vi "SC Pick Deploy.vi"(4 "projects":T1(array[cluster]), 5 "copy":string, 6 "local":i32=-1, 7 "struck":bool[](array[boolean]), 8 "symbols":i32[](array[numeric]), 9 "items":string[](array[string]), 10 "window title":string="Deploy History", 11 "current":i32=-1) -> (0 "project":i32=-1, 1 "index":i32=-1, 2 "chosen?":bool, 3 "action":string)   [LabVIEW 2023]
doc: "Shows a window listing the items, each with its symbol, the current one in bold, the local one in italics and struck ones struck through, with Check Out, Redeploy and Cancel buttons. Double-clicking an item or selecting it and clicking Redeploy returns its index; action is redeploy or check out (with chosen? and index), delete project (the Delete Project button), open copy (Open Project, shown when copy names the shown project's local .lvproj), fetch project (Fetch Project, shown instead of Delete Project when there's no local copy), or empty. chosen? is false when the user cancels or closes the window."
panel:
  in  "Fetch Project":bool
  in  "Open Project":bool
  in  "Delete Project":bool
  in  "Project":u16(ring)
  in  "Check Out":bool
  in  "Cancel":bool
  in  "Redeploy":bool
  in  "Deploys":i32(listbox)=-1
  out "check out?":bool
  out "delete project?":bool
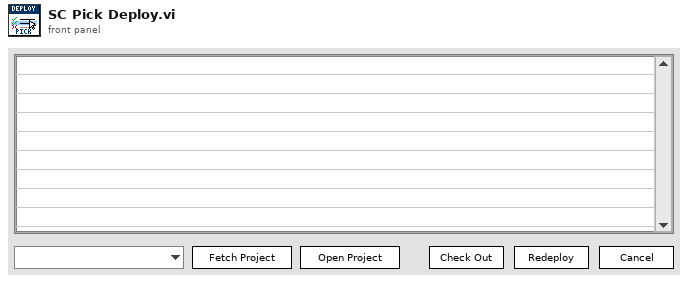
[diagram p1: front panel]
types:
  T1 = cluster{"name":string, "running":bool, "local copy":bool}[]
  T2 = typedef "LVRectTypeDef.ctl" = cluster{"Left":i16, "Top":i16, "Right":i16, "Bottom":i16}
  T3 = typedef "LVPositionTypeDef.ctl" = cluster{"Left":i32, "Top":i32}
  T4 = cluster{"name":string, "running":bool, "local copy":bool}
  T5 = typedef "LVPoint32TypeDef.ctl" = cluster{"Horizontal":i32, "Vertical":i32}
  T6 = typedef "LVRowAndColumnTypeDef.ctl" = cluster{"Row":i32, "Column":i32}
  T7 = typedef "LVPointTypeDef.ctl" = cluster{"Horizontal":i16, "Vertical":i16}
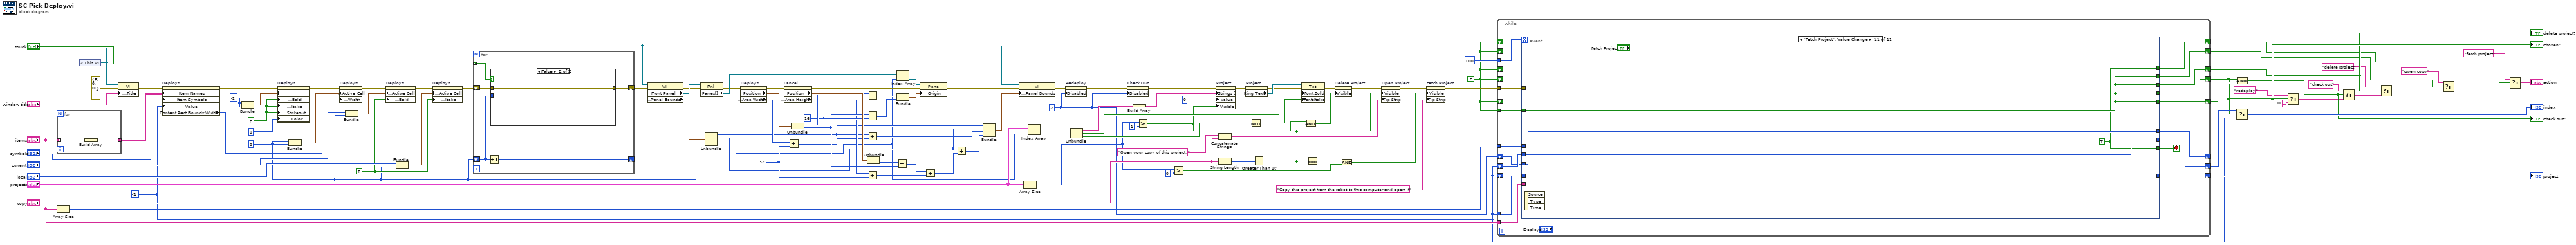
[diagram p0: block diagram]
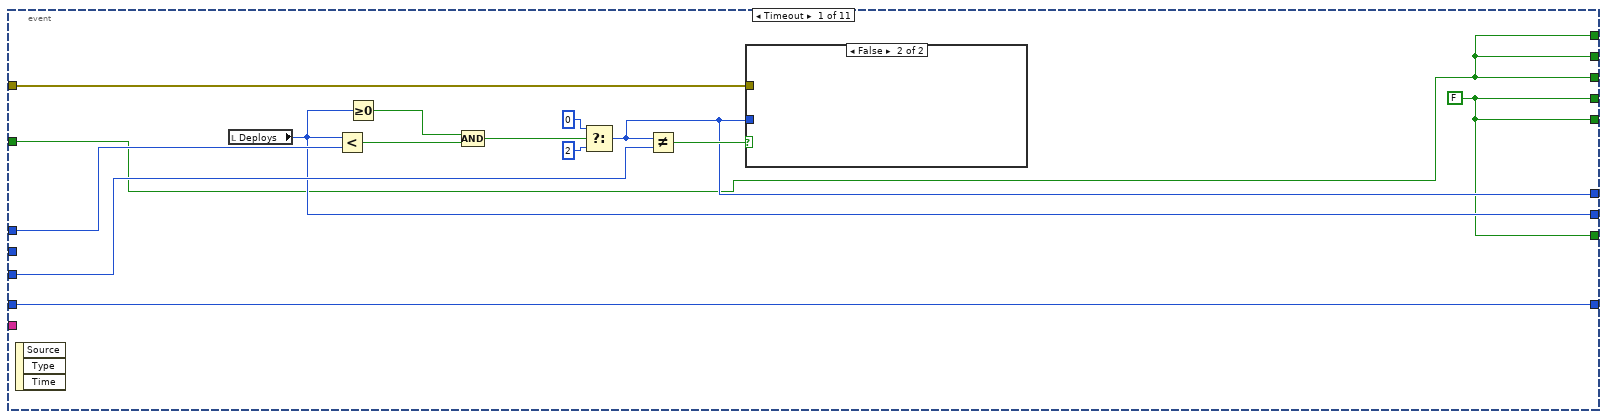
[diagram p2: hidden frame]
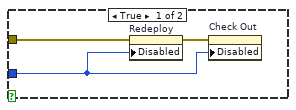
[diagram p3: hidden frame]
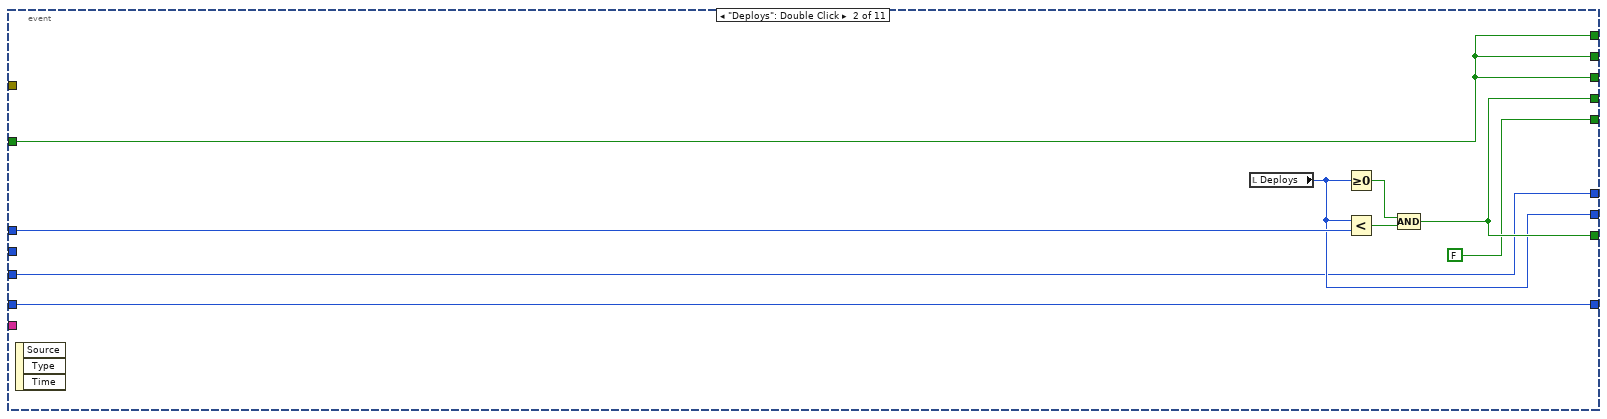
[diagram p4: hidden frame]
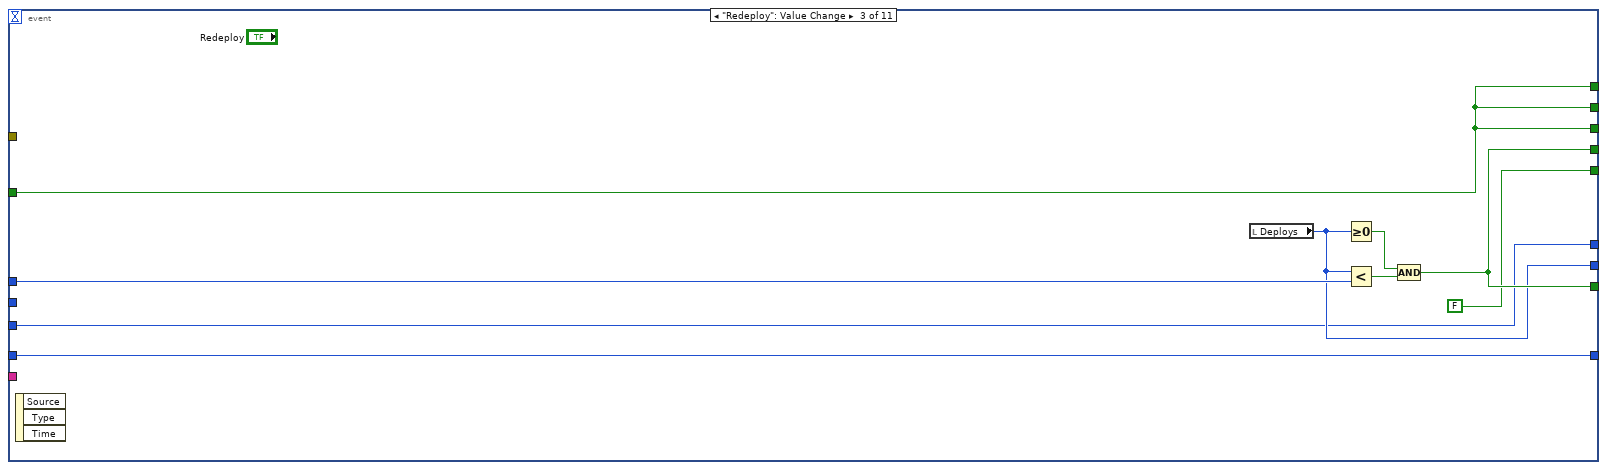
[diagram p5: hidden frame]
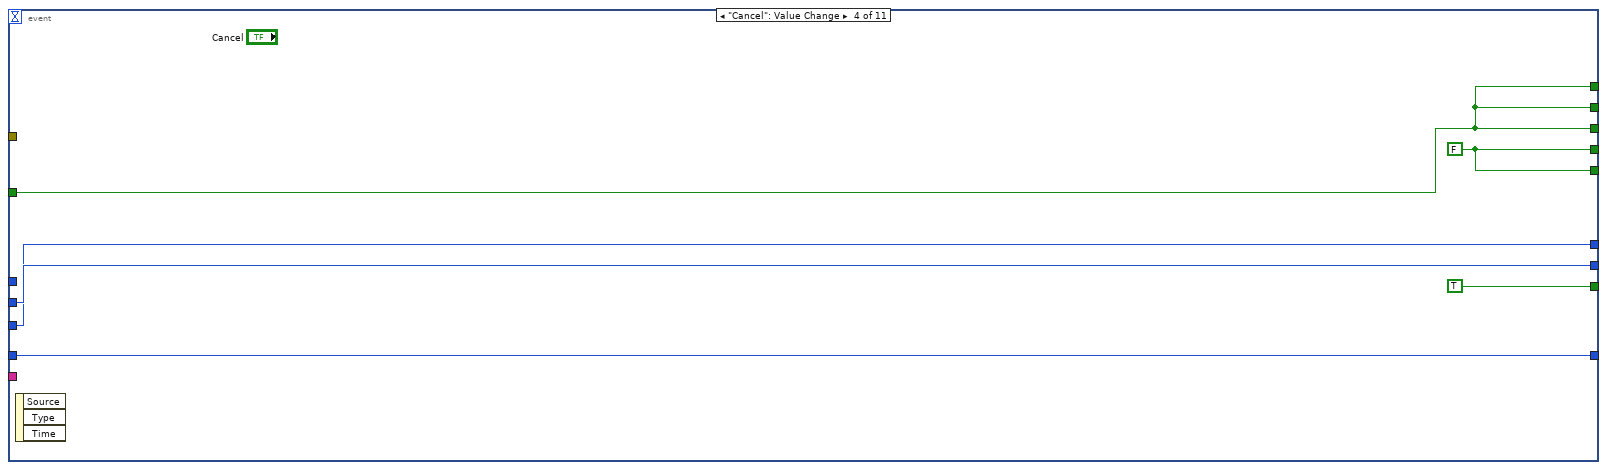
[diagram p6: hidden frame]
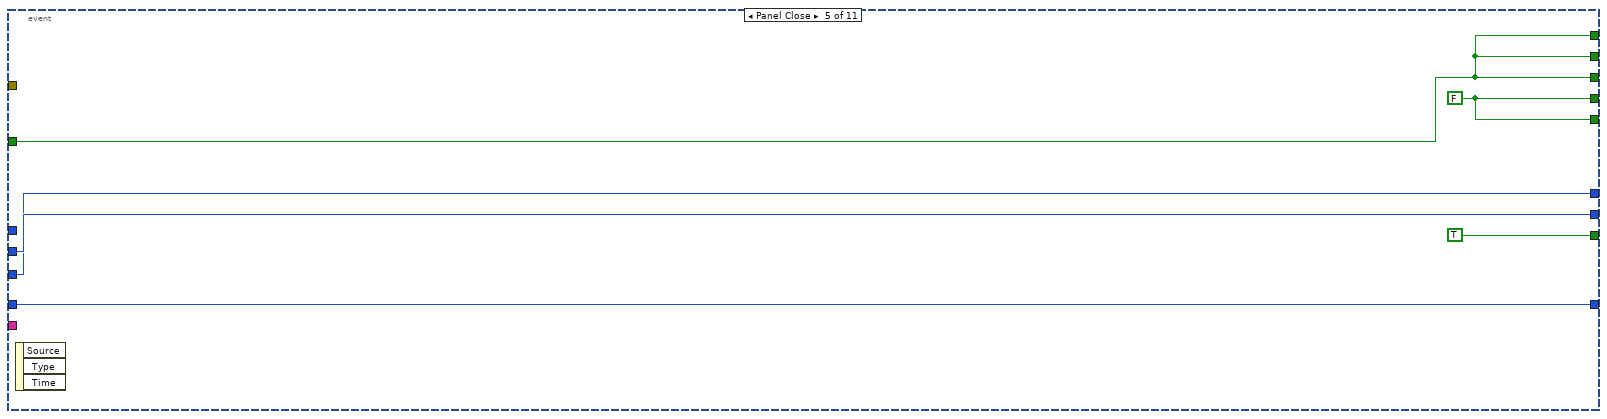
[diagram p7: hidden frame]
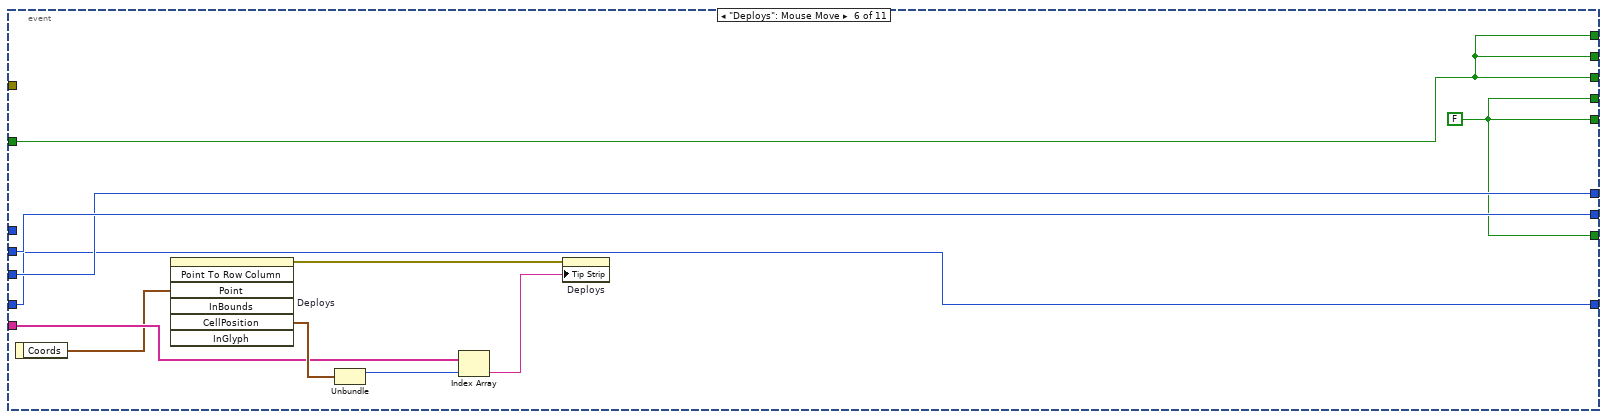
[diagram p8: hidden frame]
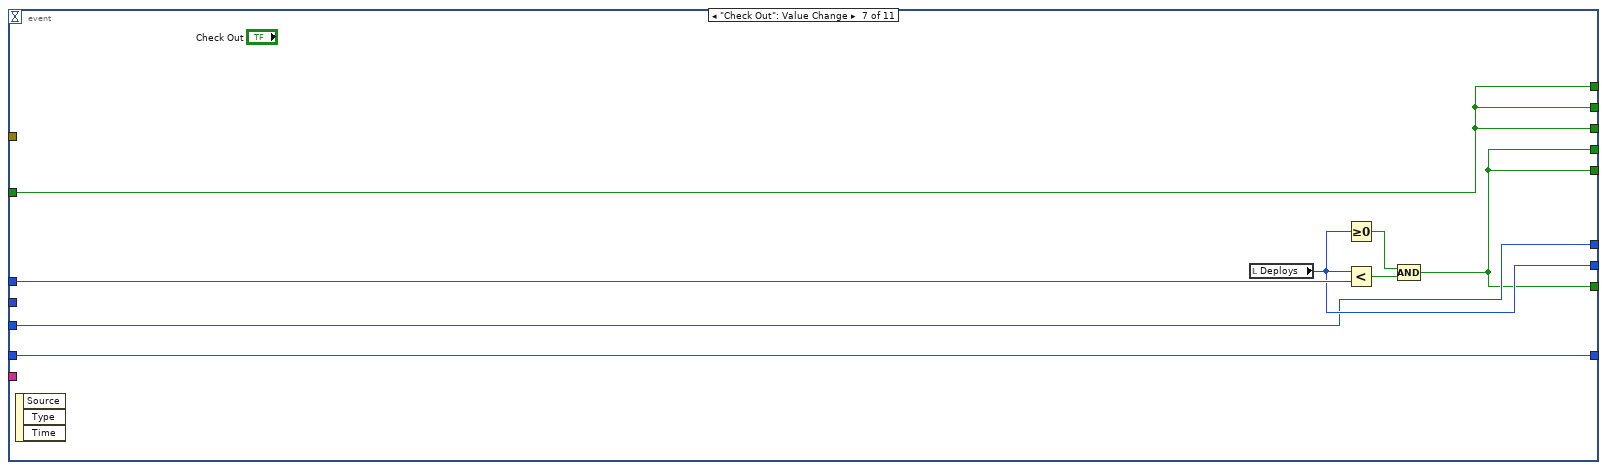
[diagram p9: hidden frame]
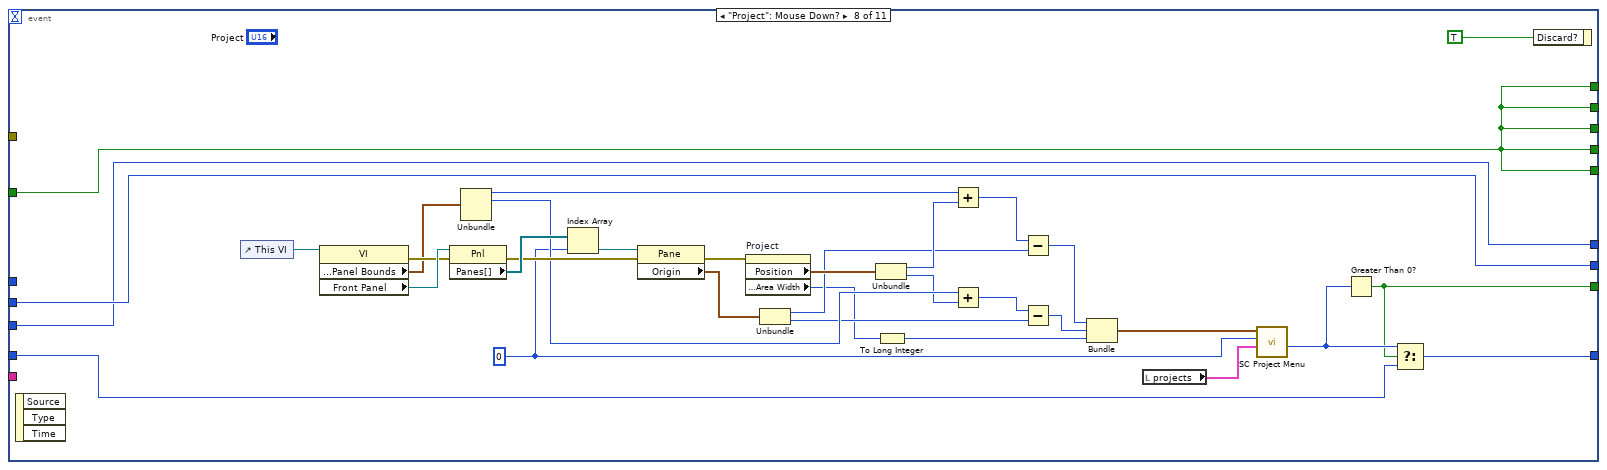
[diagram p10: hidden frame]
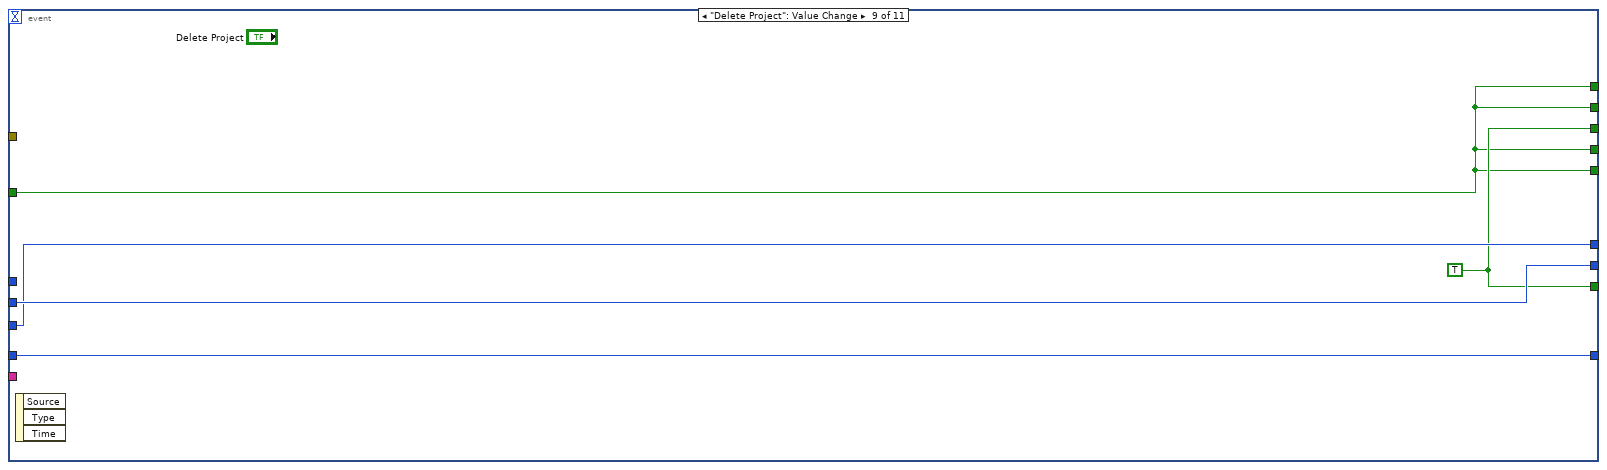
[diagram p11: hidden frame]
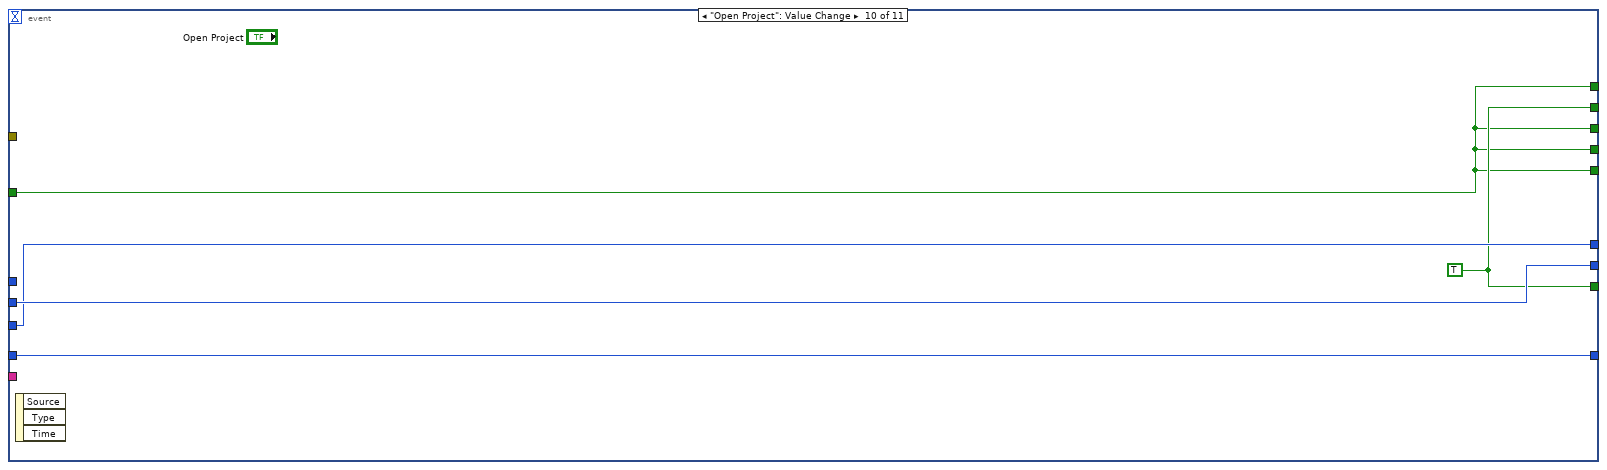
[diagram p12: hidden frame]
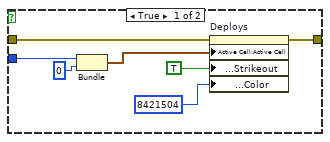
[diagram p13: hidden frame]
diagram:
  w22 = FALSE
  w74 = 32
  w81 = 16
  w94 = TRUE
  w55 = 0
  w105 = FALSE
  w108 = -2
  w21 = u8 2
  w19 = -1
  n1 = for {
    tunnel: "items" -> [w115] mode=indexing
    tunnel: [w114] -> w110 mode=indexing
    n2 = Build Array(w115) -> (w114:string[])
  }
  n3 = Array Size(array="items") -> (size(s)=w27:i32)
  n4 = control-ref of="This VI"() -> (w62:refnum<vi>)
  n5 = property class="VI"(reference=w62, error in=errorcluster {"status"=FALSE, "code"=0, "source"=""}, "Front Panel Window:Title"="window title") -> (error out=w111:errorcluster)  [unwired: 1 out]
  n6 = property on="Deploys" class="MCListbox (strict)"(error in=w111, "Item Names"=w110, "Item Symbols"="symbols", "Value"=w19) -> (error out=w107:errorcluster, "Content Rect Bounds:Width"=w100:i32)  [unwired: 1 in, 1 out]
  n7 = Bundle(w108, w108) -> (w106:cluster{i32, i32})  [unwired: 1 in]
  n8 = property on="Deploys" class="MCListbox (strict)"(error in=w107, "Active Cell:Active Cell"=w106, "Active Cell:Cell Font:Bold"=w105, "Active Cell:Cell Font:Italic"=w105, "Active Cell:Cell Font:Strikeout"=w105, "Active Cell:Cell Font:Color"=u32 0) -> (error out=w102:errorcluster)  [unwired: 1 in, 1 out]
  n9 = Bundle(w55, w55) -> (w101:cluster{i32, i32})  [unwired: 1 in]
  n10 = property on="Deploys" class="MCListbox (strict)"(error in=w102, "Active Cell:Active Cell"=w101, "Active Cell:Cell Size:Width"=w100) -> (error out=w99:errorcluster)  [unwired: 1 in, 1 out]
  n11 = Bundle("current"="current", w55) -> (w98:cluster{"current":i32, i32})  [unwired: 1 in]
  n12 = property on="Deploys" class="MCListbox (strict)"(error in=w99, "Active Cell:Active Cell"=w98, "Active Cell:Cell Font:Bold"=w94) -> (error out=w96:errorcluster)  [unwired: 1 in, 1 out]
  n13 = Bundle("local"="local", w55) -> (w95:cluster{"local":i32, i32})  [unwired: 1 in]
  n14 = property on="Deploys" class="MCListbox (strict)"(error in=w96, "Active Cell:Active Cell"=w95, "Active Cell:Cell Font:Italic"=w94) -> (error out=w92:errorcluster)  [unwired: 1 in, 1 out]
  n15 = for {
    tunnel: "struck" -> [w116] mode=indexing
    shift-right: [w120] -> _
    shift-left: w55 -> [w119]
    shift-right: [w117] -> w91
    shift-left: w92 -> [w118]
    n16 = Increment(x=w119) -> (x+1=w120:i32)
    n17 = case shown="False" w116 {
      tunnel: w119 -> [w127 _]
      tunnel: w118 -> [w125 w128]
      tunnel: [w121 w128] -> w117
      frame True {
        n18 = Bundle(w127, 0) -> (w124:cluster{i32, i32})  [unwired: 1 in]
        n19 = property on="Deploys" class="MCListbox (strict)"(error in=w125, "Active Cell:Active Cell"=w124, "Active Cell:Cell Font:Strikeout"=TRUE, "Active Cell:Cell Font:Color"=u32 8421504) -> (error out=w121:errorcluster)  [unwired: 1 in, 1 out]
      }
      frame False {
      }
    }
  }
  n20 = property class="VI"(reference=w62, error in=w91) -> (error out=w89:errorcluster, "Front Panel"=w90:refnum<vi>, "Front Panel Window:Panel Bounds"=w83:T2)  [unwired: 1 out]
  n21 = property class="Pnl"(reference=w90, error in=w89) -> (error out=w87:errorcluster, "Panes[]"=w88:refnum<vi>[])  [unwired: 1 out]
  n22 = Unbundle(w83) -> ("Left"=w69:i16, "Top"=w68:i16)  [unwired: 2 out]
  n23 = property on="Deploys" class="MCListbox (strict)"(error in=w87) -> (error out=w86:errorcluster, "Position"=w85:T3, "Bounds:Area Width"=w78:u32)  [unwired: 1 in, 1 out]
  n24 = property on="Cancel" class="Bool"(error in=w86) -> (error out=w64:errorcluster, "Position"=w84:T3, "Bounds:Area Height"=w75:u32)  [unwired: 1 in, 1 out]
  n25 = Add(x=w78, y=w74) -> (x+y=w71:u32)
  n26 = Unbundle(w85) -> ("Left"=w82:i32, "Top"=w76:i32)
  n27 = Subtract(x=w82, y=w81) -> (x-y=w80:i32)
  n28 = Subtract(x=w76, y=w81) -> (x-y=w79:i32)
  n29 = Add(x=w69, y=w71) -> (x+y=w67:u32)
  n30 = Add(x=w75, y=w74) -> (x+y=w72:u32)
  n31 = Unbundle(w84) -> ("Top"=w77:i32)  [unwired: 1 out]
  n32 = Subtract(x=w77, y=w76) -> (x-y=w73:i32)
  n33 = Index Array(array=w88, index=w55) -> (element=w65:refnum<vi>)
  n34 = Bundle(w80, w79) -> (w63:cluster{i32, i32})  [unwired: 1 in]
  n35 = property class="Pane"(reference=w65, error in=w64, "Origin"=w63) -> (error out=w61:errorcluster)  [unwired: 1 out]
  n36 = Add(x=w73, y=w72) -> (x+y=w70:u32)
  n37 = Add(x=w68, y=w70) -> (x+y=w66:u32)
  n38 = Bundle("Left"=w69, "Top"=w68, w67, w66) -> (w60:cluster{"Left":i16, "Top":i16, u32, u32})  [unwired: 1 in]
  n39 = property class="VI"(reference=w62, error in=w61, "Front Panel Window:Panel Bounds"=w60) -> (error out=w59:errorcluster)  [unwired: 1 out]
  n40 = Array Size(array="projects") -> (size(s)=w34:i32)
  n41 = Index Array(array="projects", index=w55) -> (element=w54:T4)
  n42 = property on="Redeploy" class="Bool"(error in=w59, "Disabled"=w21) -> (error out=w58:errorcluster)  [unwired: 1 in, 1 out]
  n43 = Unbundle(w54) -> ("name"=w53:string, "running"=w49:bool, "local copy"=w52:bool)
  n44 = property on="Check Out" class="Bool"(error in=w58, "Disabled"=w21) -> (error out=w47:errorcluster)  [unwired: 1 in, 1 out]
  n45 = Build Array(w53) -> (w46:string[])
  n46 = Greater?(x=w34, y=1) -> (0:w37:bool)
  n47 = Greater?(x=w34, y=0) -> (0:w31:bool)
  n48 = property on="Project" class="Ring (strict)"(error in=w47, "Strings []"=w46, "Value"=u16 0, "Visible"=w37) -> (error out=w44:errorcluster)  [unwired: 1 in, 1 out]
  n49 = Concatenate Strings("Open your copy of this project: ", "copy") -> (w38:string)
  n50 = String Length(string="copy") -> (length=w42:i32)
  n51 = property on="Project" class="Ring (strict)"(error in=w44) -> (error out=w50:errorcluster, "Ring Text"=w51:refnum<vi>)  [unwired: 1 in, 1 out]
  n52 = Not(x=w52) -> (.not. x?=w48:bool)
  n53 = Greater Than 0?(x=w42) -> (x > 0?=w35:bool)
  n54 = property class="Txt"(reference=w51, error in=w50, "Font:Bold"=w49, "Font:Italic"=w48) -> (error out=w43:errorcluster)  [unwired: 1 out]
  n55 = And(x=w37, y=w35) -> (x .and. y?=w36:bool)
  n56 = Not(x=w35) -> (.not. x?=w32:bool)
  n57 = property on="Delete Project" class="Bool"(error in=w43, "Visible"=w36) -> (error out=w39:errorcluster)  [unwired: 1 in, 1 out]
  n58 = And(x=w32, y=w31) -> (x .and. y?=w29:bool)
  n59 = property on="Open Project" class="Bool"(error in=w39, "Visible"=w35, "Tip Strip"=w38) -> (error out=w30:errorcluster)  [unwired: 1 in, 1 out]
  n60 = property on="Fetch Project" class="Bool"(error in=w30, "Visible"=w29, "Tip Strip"="Copy this project from the robot to this computer and open it") -> (error out=w26:errorcluster)  [unwired: 1 in, 1 out]
  n61 = while {
    tunnel: w27 -> [w145]
    tunnel: w26 -> [w143]
    tunnel: 100 -> [w129]
    tunnel: "items" -> [w141]
    tunnel: w19 -> [w137]
    tunnel: w22 -> [w136]
    shift-right: [w139] -> w20
    shift-left: w19 -> [w144]
    shift-right: [w140] -> w16
    shift-left: w22 -> [_]
    shift-right: [w135] -> w17
    shift-left: w22 -> [_]
    shift-right: [w134] -> w23
    shift-left: w19 -> [_]
    shift-right: [w133] -> w10
    shift-left: w22 -> [_]
    shift-right: [w131] -> w4
    shift-left: w22 -> [_]
    shift-right: [w132] -> w7
    shift-left: w22 -> [_]
    shift-right: [w138] -> _
    shift-left: w21 -> [w142]
    stop <- w130 stop-if-true
    n62 = event shown="[10] \"Fetch Project\": Value Change" {
      selector: _ -> [_ _ _ _ _ _ _ _ _ _ _]
      dyn-events: _ -> [_ _ _ _ _ _ _ _ _ _ _]
      timeout: w129 -> [_ _ _ _ _ _ _ _ _ _ _]
      tunnel: w145 -> [w159 w171 w180 _ _ _ w211 _ _ _ _]
      tunnel: w144 -> [_ _ _ w185 w191 w198 _ w216 w249 w254 w259]
      tunnel: w143 -> [w152 _ _ _ _ _ _ _ _ _ _]
      tunnel: w142 -> [w153 w166 w175 w184 w190 w197 w207 w215 w248 w253 w258]
      tunnel: w141 -> [_ _ _ _ _ w202 _ _ _ _ _]
      tunnel: [w148 w168 w177 TRUE TRUE w196 w206 w217 w246 w251 w255] -> w130
      tunnel: [w148 w168 w177 w183 w189 w196 w206 w213 w245 w250 w256] -> w140
      tunnel: [w150 w167 w176 w185 w191 w198 w208 w216 w249 w254 w259] -> w139
      tunnel: [w149 w166 w175 w184 w190 w197 w207 w215 w248 w253 w258] -> w138
      tunnel: w137 -> [w147 w164 w173 w182 w188 w195 w205 w218 w247 w252 w257]
      tunnel: w136 -> [w146 w163 w172 w181 w187 w194 w204 w213 w245 w250 w256]
      tunnel: [w148 FALSE FALSE w183 w189 w196 w206 w213 w245 w250 w256] -> w135
      tunnel: [w147 w164 w173 w182 w188 w195 w205 w214 w247 w252 w257] -> w134
      tunnel: [w146 w163 w172 w181 w187 w194 w204 w213 w246 w250 w256] -> w133
      tunnel: [w146 w163 w172 w181 w187 w194 w204 w213 w245 w251 w256] -> w132
      tunnel: [w146 w163 w172 w181 w187 w194 w204 w213 w245 w250 w255] -> w131
      event Timeout {
        w148 = FALSE
        n63 = event-data() -> ()  [unwired: 1 in, 3 out]
        n64 = local read "Deploys"() -> (w150:i32)
        n65 = Less?(x=w150, y=w159) -> (x < y?=w157:bool)
        n66 = Greater Or Equal To 0?(x=w150) -> (x >= 0?=w158:bool)
        n67 = Compound Arithmetic op=AND(w158, w157) -> (w156:bool)
        n68 = Select(t=u8 0, s=w156, f=u8 2) -> (s? t:f=w149:u8)
        n69 = Not Equal?(x=w149, y=w153) -> (x != y?=w151:bool)
        n70 = case shown="False" w151 {
          tunnel: w149 -> [w160 _]
          tunnel: w152 -> [w162 _]
          frame True {
            n71 = property on="Redeploy" class="Bool"(error in=w162, "Disabled"=w160) -> (error out=w161:errorcluster)  [unwired: 1 in, 1 out]
            n72 = property on="Check Out" class="Bool"(error in=w161, "Disabled"=w160) -> ()  [unwired: 1 in, 2 out]
          }
          frame False {
          }
        }
      }
      event "Deploys": Double Click {
        n73 = event-data() -> ()  [unwired: 1 in, 3 out]
        n74 = local read "Deploys"() -> (w167:i32)
        n75 = Greater Or Equal To 0?(x=w167) -> (x >= 0?=w170:bool)
        n76 = Less?(x=w167, y=w171) -> (x < y?=w169:bool)
        n77 = Compound Arithmetic op=AND(w170, w169) -> (w168:bool)
      }
      event "Redeploy": Value Change {
        n78 = event-data() -> ()  [unwired: 1 in, 3 out]
        n79 = local read "Deploys"() -> (w176:i32)
        n80 = Greater Or Equal To 0?(x=w176) -> (x >= 0?=w179:bool)
        n81 = Less?(x=w176, y=w180) -> (x < y?=w178:bool)
        n82 = Compound Arithmetic op=AND(w179, w178) -> (w177:bool)
      }
      event "Cancel": Value Change {
        w183 = FALSE
        n83 = event-data() -> ()  [unwired: 1 in, 3 out]
      }
      event Panel Close {
        w189 = FALSE
        n84 = event-data() -> ()  [unwired: 1 in, 3 out]
      }
      event "Deploys": Mouse Move {
        w196 = FALSE
        n85 = event-data() -> ("Coords"=w193:T5)  [unwired: 1 in]
        n86 = invoke on="Deploys" class="MCListbox (strict)" method="Point To Row Column"("Point"=w193) -> (error out=w200:errorcluster, "CellPosition"=w203:T6)  [unwired: 6 in, 5 out]
        n87 = Unbundle(w203) -> ("Row"=w201:i32)  [unwired: 1 out]
        n88 = Index Array(array=w202, index=w201) -> (element=w199:string)
        n89 = property on="Deploys" class="MCListbox (strict)"(error in=w200, "Tip Strip"=w199) -> ()  [unwired: 1 in, 2 out]
      }
      event "Check Out": Value Change {
        n90 = event-data() -> ()  [unwired: 1 in, 3 out]
        n91 = local read "Deploys"() -> (w208:i32)
        n92 = Greater Or Equal To 0?(x=w208) -> (x >= 0?=w210:bool)
        n93 = Less?(x=w208, y=w211) -> (x < y?=w209:bool)
        n94 = Compound Arithmetic op=AND(w210, w209) -> (w206:bool)
      }
      event "Project": Mouse Down? {
        w221 = 0
        n95 = event-data() -> ()  [unwired: 1 in, 3 out]
        n96 = control-ref of="This VI"() -> (w244:refnum<vi>)
        n97 = property class="VI"(reference=w244) -> (error out=w242:errorcluster, "Front Panel Window:Panel Bounds"=w237:T2, "Front Panel"=w243:refnum<vi>)  [unwired: 1 in, 1 out]
        n98 = property class="Pnl"(reference=w243, error in=w242) -> (error out=w239:errorcluster, "Panes[]"=w241:refnum<vi>[])  [unwired: 1 out]
        n99 = Unbundle(w237) -> ("Left"=w234:i16, "Top"=w230:i16)  [unwired: 2 out]
        n100 = Index Array(array=w241, index=w221) -> (element=w240:refnum<vi>)
        n101 = property class="Pane"(reference=w240, error in=w239) -> (error out=w238:errorcluster, "Origin"=w236:T7)  [unwired: 1 out]
        n102 = property on="Project" class="Ring (strict)"(error in=w238) -> ("Position"=w235:T3, "Bounds:Area Width"=w226:u32)  [unwired: 1 in, 2 out]
        n103 = Unbundle(w236) -> ("Horizontal"=w231:i16, "Vertical"=w227:i16)
        n104 = Unbundle(w235) -> ("Left"=w233:i32, "Top"=w229:i32)
        n105 = To Long Integer(number=w226) -> (32bit integer=w223:i32)
        n106 = Add(x=w234, y=w233) -> (x+y=w232:i32)
        n107 = Add(x=w230, y=w229) -> (x+y=w228:i32)
        n108 = Subtract(x=w232, y=w231) -> (x-y=w225:i32)
        n109 = Subtract(x=w228, y=w227) -> (x-y=w224:i32)
        n110 = Bundle(w225, w224, w223) -> (w220:cluster{i32, i32, i32})  [unwired: 1 in]
        n111 = local read "projects"() -> (w222:T1)
        n112 = call "SC Project Menu.vi"("projects"=w222, "selected"=w221, "position"=w220) -> ("index"=w219:i32)  [unwired: 8 in]
        n113 = Greater Than 0?(x=w219) -> (x > 0?=w217:bool)
        n114 = Select(t=w219, s=w217, f=w218) -> (s? t:f=w214:i32)
        n115 = event-data("Discard?"=TRUE) -> ()  [unwired: 1 in, 1 out]
      }
      event "Delete Project": Value Change {
        w246 = TRUE
        n116 = event-data() -> ()  [unwired: 1 in, 3 out]
      }
      event "Open Project": Value Change {
        w251 = TRUE
        n117 = event-data() -> ()  [unwired: 1 in, 3 out]
      }
      event "Fetch Project": Value Change {
        w255 = TRUE
        n118 = event-data() -> ()  [unwired: 1 in, 3 out]
      }
    }
  }
  "chosen?" <- w16
  "project" <- w23
  "delete project?" <- w10
  n119 = Select(t=w20, s=w16, f=w19) -> (s? t:f=→"index":i32)
  n120 = Compound Arithmetic op=AND(w16, w17) -> (w13:bool)
  "check out?" <- w13
  n121 = Select(t="redeploy", s=w16, f="") -> (s? t:f=w11:string)
  n122 = Select(t="check out", s=w13, f=w11) -> (s? t:f=w8:string)
  n123 = Select(t="delete project", s=w10, f=w8) -> (s? t:f=w5:string)
  n124 = Select(t="open copy", s=w7, f=w5) -> (s? t:f=w2:string)
  n125 = Select(t="fetch project", s=w4, f=w2) -> (s? t:f=→"action":string)
